vi "Resolve Headers.vi"(7 "REST Client in":refnum<class "REST Client.lvclass">, 11 "headers in":T1[](array[typedef])) -> (3 "headers out":T1[](array[typedef]))   [LabVIEW 2020, in "REST Client.lvlib" / "REST Client.lvclass"]
uses:
  REST Client.lvclass
  HTTP Header.ctl
  <vilib>/NI/Advanced HTTP Client/Header--Combo Box.ctl
  REST Client.lvclass/REST Client.ctl
  <vilib>/NI/Advanced HTTP Client/Session.lvclass
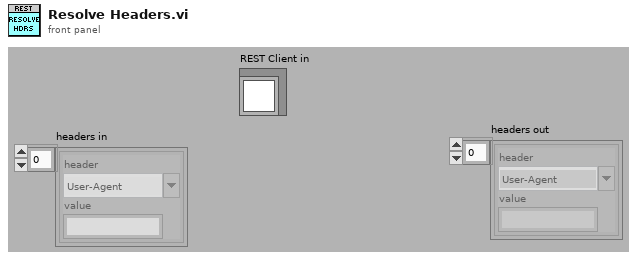
[diagram p1: front panel]
types:
  T1 = typedef "REST Client.lvlib/REST Client.lvclass/HTTP Header.ctl" = cluster{"header":T2, "value":string}
  T2 = typedef "lib_NI_Advanced HTTP Client.lvlib/Session.lvclass/Header--Combo Box.ctl" = string
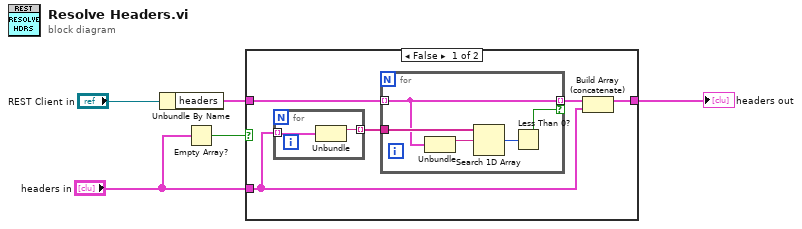
[diagram p0: block diagram]
diagram:
  n1 = Unbundle By Name("REST Client in") -> ("headers"=w1:cluster{"header":string, "value":string}[])
  n2 = Empty Array?(array="headers in") -> (empty?=w2:bool)
  n3 = case shown="False" w2 {
    tunnel: "headers in" -> [w6 _]
    tunnel: w1 -> [w10 w18]
    tunnel: [w9 w18] -> w3
    frame False {
      n4 = for {
        tunnel: w6 -> [w11] mode=indexing
        tunnel: [w12] -> w7 mode=indexing
        n5 = Unbundle(w11) -> ("header"=w12:T2)  [unwired: 1 out]
      }
      n6 = for {
        tunnel: w10 -> [w14] mode=indexing
        tunnel: w7 -> [w17]
        tunnel: [w14] -> w8 mode=indexing if=w13
        n7 = Unbundle(w14) -> ("header"=w16:string)  [unwired: 1 out]
        n8 = Search 1D Array(1D array=w17, element=w16) -> (index of element=w15:i32)  [unwired: 1 in]
        n9 = Less Than 0?(x=w15) -> (x < 0?=w13:bool)
      }
      n10 = Build Array (concatenate)(w8, w6) -> (w9:T1[])
    }
    frame True {
    }
  }
  "headers out" <- w3
